vi "Set PWM Dutty Cycle.Software.vi"(8 "error in (no error)":errorcluster, 9 "PWM Timing":cluster{"PWM Range":u32, "PWM Data":u32}, 10 "Duty Cycle (0-1)":dbl=0.5, 11 "RPi PWM Pin in":T1) -> (0 "error out":errorcluster, 3 "RPi PWM Pin out":T1=enum."GPIO2_I2C1_SDA_Pin3")   [LabVIEW 2020, in "wiringPi.lvlib"]
doc: "<b>_______________________________________________________________</b>\n** Author: Juan José Villacorta\n** LabVIEW wrapper for C library <b> wiringPi </b>,\n** https://github.com/WiringPi/WiringPi\n<b>_______________________________________________________________</b>\n\nConfigure a PWM dutty-cycle. Set 0 to stop PWM"
uses:
  wiringPi.lvlib
  Type Defs/GPIO Pins.ctl
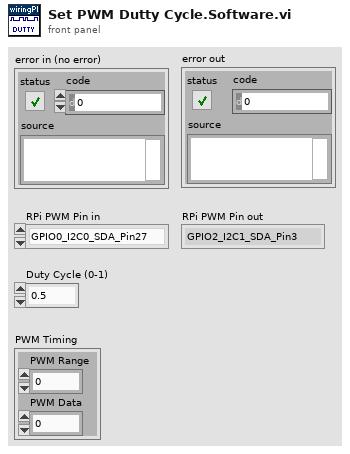
[diagram p1: front panel]
types:
  T1 = typedef "wiringPi.lvlib/GPIO Pins.ctl" = enum32{"GPIO0_I2C0_SDA_Pin27", "GPIO1_I2C0_SDA1_Pin28", "GPIO2_I2C1_SDA_Pin3", "GPIO3_I2C1_SCL_Pin5", "GPIO4_GPCLK0_Pin7", "GPIO5_GPCLK1_Pin29", "GPIO6_GPCLK2_Pin31", "GPIO7_SPI_CE1_N_Pin26", "GPIO8_SPI_CE0_N_Pin24", "GPIO9_SPI0_MISO_Pin21", "GPIO10_SPI0_MOSI_Pin19", "GPIO11_SPI0_CLK_Pin23", "GPIO12_PWM0_Pin32", "GPIO13_PWM1_Pin33", "GPIO14_TXD0_Pin8", "GPIO15_RXD0_Pin10", "GPIO16_Pin36", "GPIO17_Pin11", "GPIO18_PWM0_Pin12", "GPIO19_PWM1_Pin35", "GPIO20_GPCLK0_Pin38", "GPIO21_GPCLK1_Pin40", "GPIO22_Pin15", "GPIO23_Pin16", "GPIO24_Pin18", "GPIO25_Pin22", "GPIO26_Pin37", "GPIO27_Pin13"}
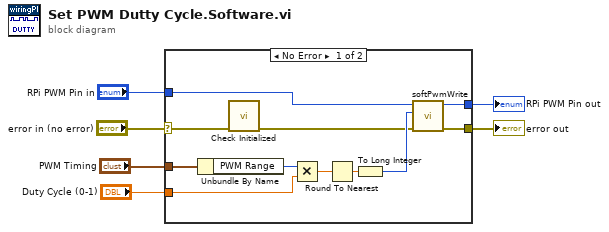
[diagram p0: block diagram]
diagram:
  n1 = case shown="No Error" "error in (no error)" {
    selector: "error in (no error)" -> [w8 w19]
    tunnel: [w12 w19] -> w5
    tunnel: "RPi PWM Pin in" -> [w9 w18]
    tunnel: "PWM Timing" -> [w17 _]
    tunnel: "Duty Cycle (0-1)" -> [w15 _]
    tunnel: [w10 w18] -> w1
    frame No Error {
      n2 = Unbundle By Name(w17) -> ("PWM Range"=w16:u32)
      n3 = call "Check Initialized.vi"("error in (no error)"=w8) -> ("error out"=w7:errorcluster)  [unwired: 10 in]
      n4 = Multiply(x=w16, y=w15) -> (x*y=w13:dbl)
      n5 = Round To Nearest(number=w13) -> (nearest integer value=w14:dbl)
      n6 = To Long Integer(number=w14) -> (32bit integer=w11:i32)
      n7 = call "softPwmWrite.vi"("error in (no error)"=w7, "Value"=w11, "RPi Pin"=w9) -> ("error out"=w12:errorcluster, "RPi Pin out"=w10:T1)  [unwired: 7 in]
    }
    frame Error {
    }
  }
  "error out" <- w5
  "RPi PWM Pin out" <- w1
